vi "Convert Numeric Register Value.vi"(8 "Signed representation":T1, 9 "Order":T2, 10 "Numeric Input":T3, 11 "Register Values":u16[](array[numeric])) -> (3 "Number out":dbl)   [LabVIEW 2026, in "Modbus.lvlib" / "Modbus.lvclass"]
uses:
  Modbus.lvclass
  Types/Numeric Data.ctl
  Types/Modbus Table.ctl
  Types/Numeric Size.ctl
  Types/Numeric Data Type.ctl
  Types/Numeric Location.ctl
  Types/Order.ctl
  Utility/Signed Representation/Types/Signed Representation.ctl
  52ccbd75-5339-40bf-91bf-28e664d3472a.vi
  8f5713fc-c990-4029-b5da-ac4b65fa98e9.vi
  8f9408a0-d04d-4472-9a21-a9ae7f5b0722.vi
  ee27a5e4-b4cd-4cb3-9cf9-9ec45526a22d.vi
  52ccbd75-5339-40bf-91bf-28e664d3472a.vi/075529c4-3756-4c35-a727-d79a570b4e4b.vi
  52ccbd75-5339-40bf-91bf-28e664d3472a.vi/f2b159a7-3f15-4c07-8087-86d897f3e084.vi
  52ccbd75-5339-40bf-91bf-28e664d3472a.vi/e7f4747e-5a28-4a2e-9592-f11bd74c8d05.vi
  52ccbd75-5339-40bf-91bf-28e664d3472a.vi/dfb42b1f-79ab-4f7c-b389-1108b947dcfb.vi
  52ccbd75-5339-40bf-91bf-28e664d3472a.vi/5f52ec6b-8d9c-4a1b-8cba-4e2f2acbbc65.vi
  52ccbd75-5339-40bf-91bf-28e664d3472a.vi/9402299f-8d08-4b56-b955-c752433d99a7.vi
  52ccbd75-5339-40bf-91bf-28e664d3472a.vi/587ca7da-2917-4b98-b856-e292118fa9d0.vi
  52ccbd75-5339-40bf-91bf-28e664d3472a.vi/d9cf77ad-bfa9-4690-bb58-8188d63c027f.vi
  52ccbd75-5339-40bf-91bf-28e664d3472a.vi/0dbe1b4e-815d-48eb-bf8e-9c4112dc030e.vi
  8f5713fc-c990-4029-b5da-ac4b65fa98e9.vi/075529c4-3756-4c35-a727-d79a570b4e4b.vi
  8f5713fc-c990-4029-b5da-ac4b65fa98e9.vi/f2b159a7-3f15-4c07-8087-86d897f3e084.vi
  8f5713fc-c990-4029-b5da-ac4b65fa98e9.vi/e7f4747e-5a28-4a2e-9592-f11bd74c8d05.vi
  8f5713fc-c990-4029-b5da-ac4b65fa98e9.vi/dfb42b1f-79ab-4f7c-b389-1108b947dcfb.vi
  8f5713fc-c990-4029-b5da-ac4b65fa98e9.vi/5f52ec6b-8d9c-4a1b-8cba-4e2f2acbbc65.vi
  8f5713fc-c990-4029-b5da-ac4b65fa98e9.vi/9402299f-8d08-4b56-b955-c752433d99a7.vi
  8f5713fc-c990-4029-b5da-ac4b65fa98e9.vi/587ca7da-2917-4b98-b856-e292118fa9d0.vi
  8f5713fc-c990-4029-b5da-ac4b65fa98e9.vi/d9cf77ad-bfa9-4690-bb58-8188d63c027f.vi
  8f5713fc-c990-4029-b5da-ac4b65fa98e9.vi/0dbe1b4e-815d-48eb-bf8e-9c4112dc030e.vi
  8f9408a0-d04d-4472-9a21-a9ae7f5b0722.vi/075529c4-3756-4c35-a727-d79a570b4e4b.vi
  8f9408a0-d04d-4472-9a21-a9ae7f5b0722.vi/f2b159a7-3f15-4c07-8087-86d897f3e084.vi
  8f9408a0-d04d-4472-9a21-a9ae7f5b0722.vi/e7f4747e-5a28-4a2e-9592-f11bd74c8d05.vi
  8f9408a0-d04d-4472-9a21-a9ae7f5b0722.vi/dfb42b1f-79ab-4f7c-b389-1108b947dcfb.vi
  8f9408a0-d04d-4472-9a21-a9ae7f5b0722.vi/5f52ec6b-8d9c-4a1b-8cba-4e2f2acbbc65.vi
  8f9408a0-d04d-4472-9a21-a9ae7f5b0722.vi/9402299f-8d08-4b56-b955-c752433d99a7.vi
  8f9408a0-d04d-4472-9a21-a9ae7f5b0722.vi/587ca7da-2917-4b98-b856-e292118fa9d0.vi
  8f9408a0-d04d-4472-9a21-a9ae7f5b0722.vi/d9cf77ad-bfa9-4690-bb58-8188d63c027f.vi
  8f9408a0-d04d-4472-9a21-a9ae7f5b0722.vi/0dbe1b4e-815d-48eb-bf8e-9c4112dc030e.vi
  ee27a5e4-b4cd-4cb3-9cf9-9ec45526a22d.vi/075529c4-3756-4c35-a727-d79a570b4e4b.vi
  ee27a5e4-b4cd-4cb3-9cf9-9ec45526a22d.vi/f2b159a7-3f15-4c07-8087-86d897f3e084.vi
  ee27a5e4-b4cd-4cb3-9cf9-9ec45526a22d.vi/e7f4747e-5a28-4a2e-9592-f11bd74c8d05.vi
  ee27a5e4-b4cd-4cb3-9cf9-9ec45526a22d.vi/dfb42b1f-79ab-4f7c-b389-1108b947dcfb.vi
  ee27a5e4-b4cd-4cb3-9cf9-9ec45526a22d.vi/5f52ec6b-8d9c-4a1b-8cba-4e2f2acbbc65.vi
  ee27a5e4-b4cd-4cb3-9cf9-9ec45526a22d.vi/9402299f-8d08-4b56-b955-c752433d99a7.vi
  ee27a5e4-b4cd-4cb3-9cf9-9ec45526a22d.vi/587ca7da-2917-4b98-b856-e292118fa9d0.vi
  ee27a5e4-b4cd-4cb3-9cf9-9ec45526a22d.vi/d9cf77ad-bfa9-4690-bb58-8188d63c027f.vi
  ee27a5e4-b4cd-4cb3-9cf9-9ec45526a22d.vi/0dbe1b4e-815d-48eb-bf8e-9c4112dc030e.vi
  Utility/Utility.lvlib
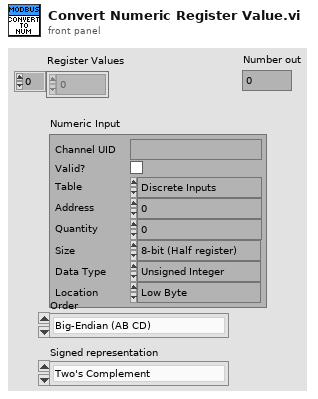
[diagram p1: front panel]
types:
  T1 = typedef "Utility.lvlib/Signed Representation.ctl" = enum16{"Two's Complement", "Offset Binary", "Sign-Magnitude", "Ones' Complement"}
  T2 = typedef "Modbus.lvlib/Modbus.lvclass/Order.ctl" = enum16{"Big-Endian (AB CD)", "Word-Swap (CD AB)", "Byte-Swap (BA DC)", "Little-Endian (DC BA)"}
  T3 = typedef "Modbus.lvlib/Modbus.lvclass/Numeric Data.ctl" = cluster{"Channel UID":string, "Valid?":bool, "Table":T4, "Address":i32, "Quantity":u16, "Size":T5, "Data Type":T6, "Location":T7}
  T4 = typedef "Modbus.lvlib/Modbus.lvclass/Modbus Table.ctl" = enum16{"Discrete Inputs", "Coils", "Input Registers", "Holding Registers"}
  T5 = typedef "Modbus.lvlib/Modbus.lvclass/Numeric Size.ctl" = enum16{"8-bit (Half register)", "16-bit (One register)", "32-bit (Two registers)", "64-bit (Four registers)"}
  T6 = typedef "Modbus.lvlib/Modbus.lvclass/Numeric Data Type.ctl" = enum16{"Unsigned Integer", "Signed Integer", "Floating Point"}
  T7 = typedef "Modbus.lvlib/Modbus.lvclass/Numeric Location.ctl" = enum16{"Low Byte", "High Byte"}
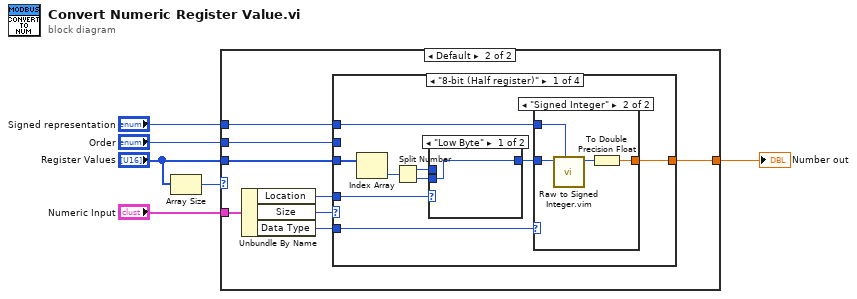
[diagram p0: block diagram]
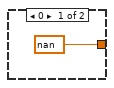
[diagram p2: hidden frame]
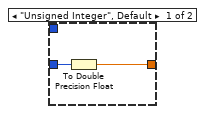
[diagram p4: hidden frame]
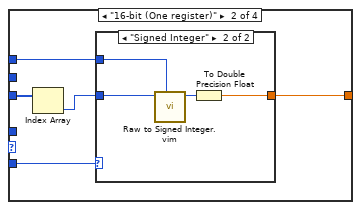
[diagram p5: hidden frame]
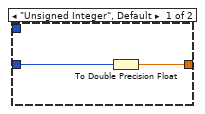
[diagram p6: hidden frame]
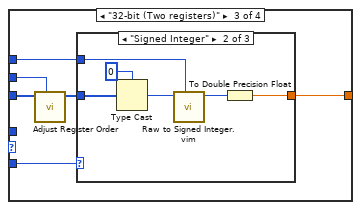
[diagram p7: hidden frame]
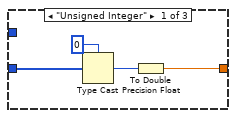
[diagram p8: hidden frame]
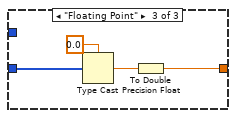
[diagram p9: hidden frame]
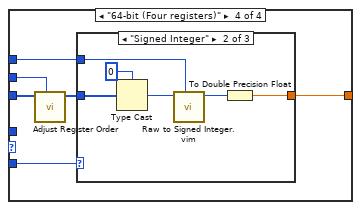
[diagram p10: hidden frame]
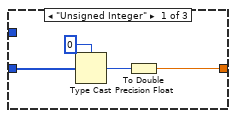
[diagram p11: hidden frame]
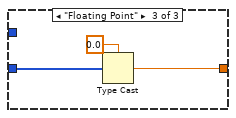
[diagram p12: hidden frame]
diagram:
  n1 = Array Size(array="Register Values") -> (size(s)=w2:i32)
  n2 = case shown="Default" w2 {
    tunnel: "Numeric Input" -> [_ w15]
    tunnel: [nan w12] -> w5
    tunnel: "Signed representation" -> [_ w11]
    tunnel: "Order" -> [_ w9]
    tunnel: "Register Values" -> [_ w8]
    frame 0 {
    }
    frame Default {
      n3 = Unbundle By Name(w15) -> ("Location"=w10:T7, "Size"=w14:T5, "Data Type"=w13:T6)
      n4 = case shown="\"8-bit (Half register)\"" w14 {
        tunnel: w8 -> [w24 w37 w45 w66]
        tunnel: w13 -> [w22 w36 w49 w69]
        tunnel: [w21 w35 w48 w68] -> w12
        tunnel: w11 -> [w20 w34 w47 w67]
        tunnel: w10 -> [w19 _ _ _]
        tunnel: w9 -> [_ _ w46 w65]
        frame "8-bit (Half register)" {
          n5 = Index Array(array=w24) -> (element=w23:u16)  [unwired: 1 in]
          n6 = Split Number(x=w23) -> (hi(x)=w18:u8, lo(x)=w17:u8)
          n7 = case shown="\"Low Byte\"" w19 {
            tunnel: w18 -> [_ w26]
            tunnel: w17 -> [w25 _]
            tunnel: [w25 w26] -> w16
            frame "Low Byte" {
            }
            frame "High Byte" {
            }
          }
          n8 = case shown="\"Signed Integer\"" w22 {
            tunnel: w16 -> [w28 w32]
            tunnel: [w27 w29] -> w21
            tunnel: w20 -> [_ w31]
            frame "Unsigned Integer", Default {
              n9 = To Double Precision Float(number=w28) -> (double precision float=w27:dbl)
            }
            frame "Signed Integer" {
              n10 = call "Raw to Signed Integer.vim"("Signed representation"=w31, "Value (raw)"=w32) -> ("Value out"=w30:i8)  [unwired: 8 in, 1 out]
              n11 = To Double Precision Float(number=w30) -> (double precision float=w29:dbl)
            }
          }
        }
        frame "16-bit (One register)" {
          n12 = Index Array(array=w37) -> (element=w33:u16)  [unwired: 1 in]
          n13 = case shown="\"Signed Integer\"" w36 {
            tunnel: w33 -> [w39 w43]
            tunnel: [w38 w40] -> w35
            tunnel: w34 -> [_ w42]
            frame "Unsigned Integer", Default {
              n14 = To Double Precision Float(number=w39) -> (double precision float=w38:dbl)
            }
            frame "Signed Integer" {
              n15 = call "Raw to Signed Integer.vim"("Signed representation"=w42, "Value (raw)"=w43) -> ("Value out"=w41:i16)  [unwired: 8 in, 1 out]
              n16 = To Double Precision Float(number=w41) -> (double precision float=w40:dbl)
            }
          }
        }
        frame "32-bit (Two registers)" {
          n17 = call "Adjust Register Order.vi"("Order"=w46, "Register Values in"=w45) -> ("Register Values out"=w44:u16[])  [unwired: 9 in]
          n18 = case shown="\"Signed Integer\"" w49 {
            tunnel: w44 -> [w51 w55 w61]
            tunnel: [w53 w57 w63] -> w48
            tunnel: w47 -> [_ w59 _]
            frame "Unsigned Integer" {
              n19 = Type Cast(type=u32 0, x=w51) -> (*(type *) &x=w50:u32)
              n20 = To Double Precision Float(number=w50) -> (double precision float=w53:dbl)
            }
            frame "Signed Integer" {
              n21 = Type Cast(type=u32 0, x=w55) -> (*(type *) &x=w54:u32)
              n22 = call "Raw to Signed Integer.vim"("Signed representation"=w59, "Value (raw)"=w54) -> ("Value out"=w58:i32)  [unwired: 8 in, 1 out]
              n23 = To Double Precision Float(number=w58) -> (double precision float=w57:dbl)
            }
            frame "Floating Point" {
              n24 = Type Cast(type=sgl 0.0, x=w61) -> (*(type *) &x=w60:sgl)
              n25 = To Double Precision Float(number=w60) -> (double precision float=w63:dbl)
            }
          }
        }
        frame "64-bit (Four registers)" {
          n26 = call "Adjust Register Order.vi"("Order"=w65, "Register Values in"=w66) -> ("Register Values out"=w64:u16[])  [unwired: 9 in]
          n27 = case shown="\"Signed Integer\"" w69 {
            tunnel: w64 -> [w71 w75 w81]
            tunnel: [w73 w77 w80] -> w68
            tunnel: w67 -> [_ w79 _]
            frame "Unsigned Integer" {
              n28 = Type Cast(type=u64 0, x=w71) -> (*(type *) &x=w70:u64)
              n29 = To Double Precision Float(number=w70) -> (double precision float=w73:dbl)
            }
            frame "Signed Integer" {
              n30 = Type Cast(type=u64 0, x=w75) -> (*(type *) &x=w74:u64)
              n31 = call "Raw to Signed Integer.vim"("Signed representation"=w79, "Value (raw)"=w74) -> ("Value out"=w78:i64)  [unwired: 8 in, 1 out]
              n32 = To Double Precision Float(number=w78) -> (double precision float=w77:dbl)
            }
            frame "Floating Point" {
              n33 = Type Cast(type=0.0, x=w81) -> (*(type *) &x=w80:dbl)
            }
          }
        }
      }
    }
  }
  "Number out" <- w5
